vi "test_GetElements.vi"() -> ()   [LabVIEW 2013]
uses:
  <vilib>/Utility/VariantDataType/UnitInfo.ctl
  <vilib>/Utility/VariantDataType/UnitType.ctl
  source/TypeDescriptor/TypeDescriptor_GetPString.vi
  source/TypeDescriptor/OpenDescriptor.lvlib
  <vilib>/Utility/VariantDataType/VariantType.lvlib
panel:
  out "has Units 2":bool
  out "has Units":bool
  out "Units":T1[](array[typedef])
  out "name":string
  out "interleaved array (noUnits)":u8[](array[numeric]) format="%.0x"
  out "interleaved array (Units)":u8[](array[numeric]) format="%.0x"
  in  "SGL":sgl[unit]=3.0
  in  "Enum":enum16{"ItemA", "Item B", "Item C#"}(ring)=enum."Item C#"
  out "enum elements":string[](array[string])
  out "cluster elements":string[](array[string])
  out "interleaved array":u8[](array[numeric]) format="%.0x"
  in  "Cluster":T3
  # "length\nxE = 14"
  # "#elements"
  # "length\nx6 = 6"
  # "length\nx6 = 7"
  # "length\nx5 = 5"
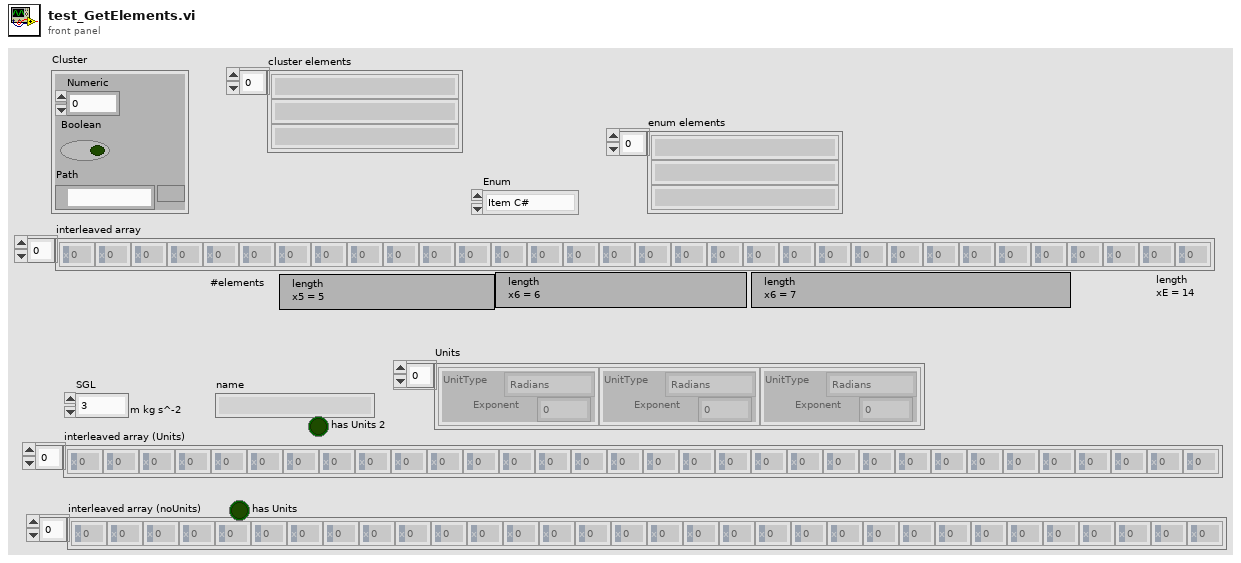
[diagram p1: front panel]
types:
  T1 = typedef "VariantType.lvlib/UnitInfo.ctl" = cluster{"UnitType":T2, "Exponent":i16}
  T2 = typedef "VariantType.lvlib/UnitType.ctl" = enum16{"Radians", "Steradians", "Seconds", "Meters", "Kilograms", "Amperes", "Kelvins", "Moles", "Candelas", "InvalidUnit"}
  T3 = cluster{"Numeric":i32, "Boolean":bool, "Path":path}
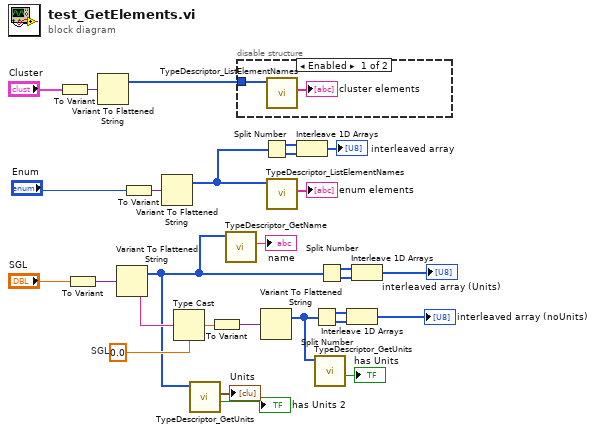
[diagram p0: block diagram]
diagram:
  w13 = sgl 0.0  # SGL
  n1 = To Variant(anything="Cluster") -> (Variant=w27:variant)
  n2 = To Variant(anything="SGL") -> (Variant=w18:variant)
  n3 = Variant To Flattened String(Variant=w27) -> (1:w26:i16[])  [unwired: 1 out]
  n4 = Variant To Flattened String(Variant=w18) -> (data string=w12:string, 1:w5:i16[])
  n5 = To Variant(anything="Enum") -> (Variant=w22:variant)
  n6 = Variant To Flattened String(Variant=w22) -> (1:w19:i16[])  [unwired: 1 out]
  n7 = Type Cast(type=w13, x=w12) -> (*(type *) &x=w10:sgl)
  n8 = call "TypeDescriptor_GetUnits.vi"("type descriptor"=w5) -> ("has Units"=→"has Units 2":bool, "Units"=→"Units":T1[])  [unwired: 8 in, 1 out]
  n9 = To Variant(anything=w10) -> (Variant=w11:variant)
  n10 = call "TypeDescriptor_GetName.vi"("type descriptor"=w5) -> ("name"=→"name":string)  [unwired: 8 in, 2 out]
  n11 = disable-structure shown="Enabled" {
    disable-tunnel: w26 -> [w30 _]
    frame Enabled {
      n12 = call "TypeDescriptor_ListElementNames.vi"("type descriptor"=w30) -> ("element names"=→"cluster elements":string[])  [unwired: 7 in, 3 out]
    }
    frame Disabled {
    }
  }
  n13 = Variant To Flattened String(Variant=w11) -> (1:w3:i16[])  [unwired: 1 out]
  n14 = Split Number(x=w19) -> (hi(x)=w25:u8[], lo(x)=w24:u8[])
  n15 = call "TypeDescriptor_ListElementNames.vi"("type descriptor"=w19) -> ("element names"=→"enum elements":string[])  [unwired: 7 in, 3 out]
  n16 = Interleave 1D Arrays(w25, w24) -> (→"interleaved array":u8[])
  n17 = Split Number(x=w3) -> (hi(x)=w9:u8[], lo(x)=w8:u8[])
  n18 = call "TypeDescriptor_GetUnits.vi"("type descriptor"=w3) -> ("has Units"=→"has Units":bool)  [unwired: 8 in, 2 out]
  n19 = Split Number(x=w5) -> (hi(x)=w15:u8[], lo(x)=w16:u8[])
  n20 = Interleave 1D Arrays(w9, w8) -> (→"interleaved array (noUnits)":u8[])
  n21 = Interleave 1D Arrays(w15, w16) -> (→"interleaved array (Units)":u8[])
